vi "Init.vi"(7 "family":string, 8 "error in":errorcluster, 9 "style":i32(ring)=1 items=["Regular"=0, "Bold"=1, "Italic"=2, "Underline"=4, "Strikeout"=8], 10 "emSize":sgl) -> (0 "error out":errorcluster, 3 "Font out":refnum<class "Font.lvclass">)   [LabVIEW 2020, in "SourceGrid.lvlib" / "Font.lvclass"]
uses:
  Font.lvclass
  Font.lvclass/Font.ctl
  System.Drawing
panel:
  in  "Font in":refnum<class "Font.lvclass">
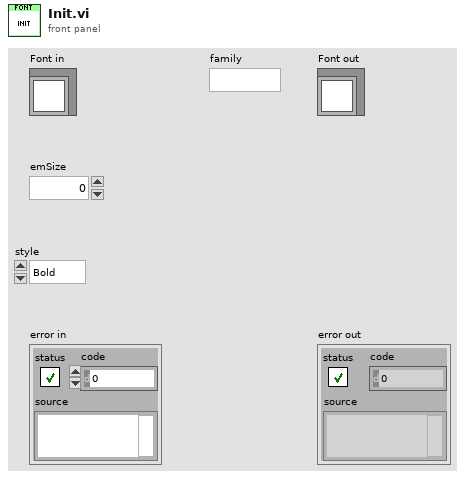
[diagram p1: front panel]
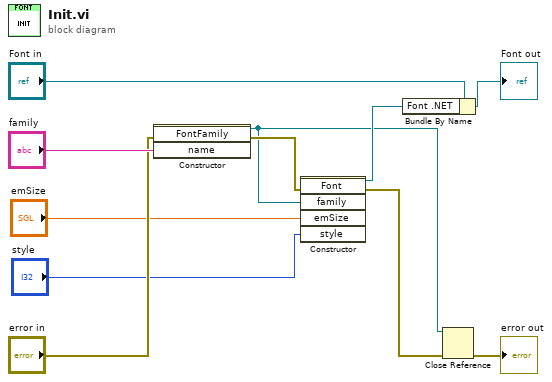
[diagram p0: block diagram]
diagram:
  n1 = constructor class="FontFamily" ("Constructor Font")(error in="error in", "name"="family") -> (reference out=w1:refnum<k24>, error out=w9:errorcluster)  [unwired: 2 in, 2 out]
  n2 = constructor class="Font" ("Constructor Font")(error in=w9, "family"=w1, "emSize"="emSize", "style"="style") -> (reference out=w3:refnum<k24>, error out=w6:errorcluster)  [unwired: 2 in, 4 out]
  n3 = Bundle By Name(cluster="Font in", "Font .NET"=w3) -> (→"Font out":refnum<class "Font.lvclass">)
  n4 = Close Reference(reference=w1, error in (no error)=w6) -> (error out=→"error out":errorcluster)
